vi "laser_constant_current_output_with_DAQ_analog_output.vi"(4 "Exit Refnum":refnum<vi>, 5 "Activate Refnum":refnum<vi>, 7 "VISA resource name":refnum<visa-resource-name>, 8 "error in (no error)":errorcluster, 9 "Current Refnum":refnum<vi>, 10 "Power Refnum":refnum<vi>, 11 "DAQmx Device":tag) -> (0 "error out":errorcluster)   [LabVIEW 2025, in "tSNIP.lvlib"]
uses:
  tSNIP.lvlib
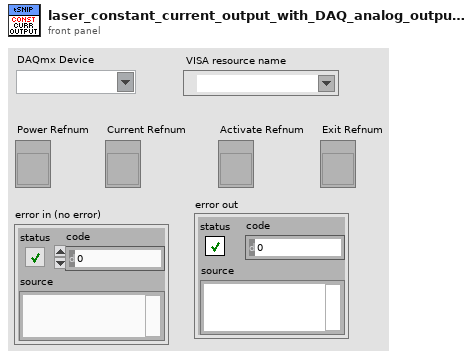
[diagram p1: front panel]
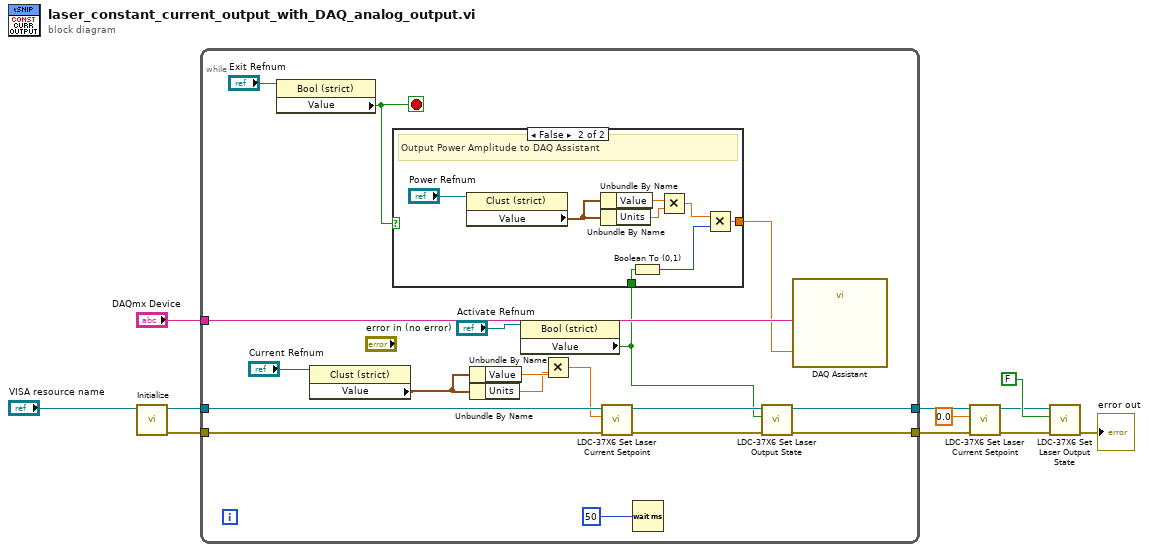
[diagram p0: block diagram]
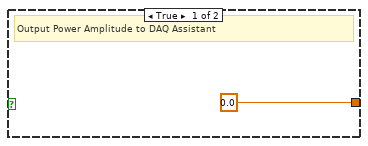
[diagram p2: hidden frame]
diagram:
  n1 = call "Initialize.vi"("VISA resource name"="VISA resource name") -> ("error out"=w9:errorcluster, "VISA resource name out"=w10:refnum<visa-resource-name>)  [unwired: 9 in]
  n2 = while {
    tunnel: w10 -> [w27]
    tunnel: w9 -> [w28]
    tunnel: [w26] -> w8
    tunnel: [w25] -> w7
    tunnel: "DAQmx Device" -> [w22]
    stop <- w12 stop-if-true
    n3 = property class="Bool (strict)"(reference="Exit Refnum") -> ("Value"=w12:bool)  [unwired: 1 in, 2 out]
    n4 = property class="Clust (strict)"(reference="Current Refnum") -> ("Value"=w13:cluster{"Value":dbl, "Units":dbl})  [unwired: 1 in, 2 out]
    n5 = Unbundle By Name(w13) -> ("Value"=w20:dbl)
    n6 = Unbundle By Name(w13) -> ("Units"=w19:dbl)
    n7 = property class="Bool (strict)"(reference="Activate Refnum") -> ("Value"=w16:bool)  [unwired: 1 in, 2 out]
    n8 = case shown="False" w12 {
      tunnel: [0.0 w37] -> w21
      tunnel: w16 -> [_ w33]
      frame True {
        # "Output Power Amplitude to DAQ Assistant"
      }
      frame False {
        # "Output Power Amplitude to DAQ Assistant"
        n9 = property class="Clust (strict)"(reference="Power Refnum") -> ("Value"=w32:cluster{"Value":dbl, "Units":dbl})  [unwired: 1 in, 2 out]
        n10 = Unbundle By Name(w32) -> ("Value"=w36:dbl)
        n11 = Unbundle By Name(w32) -> ("Units"=w35:dbl)
        n12 = Boolean To (0,1)(Boolean=w33) -> (0, 1=w38:i16)
        n13 = Multiply(x=w36, y=w35) -> (x*y=w34:dbl)
        n14 = Multiply(x=w34, y=w38) -> (x*y=w37:dbl)
      }
    }
    n15 = Multiply(x=w20, y=w19) -> (x*y=w18:dbl)
    n16 = call <instrlib>:"LDC-37X6 Set Laser Current Setpoint.vi"("VISA resource name"=w27, "Laser Current Setpoint (A)"=w18, "error in"=w28) -> ("VISA resource name out"=w24:refnum<visa-resource-name>, "error out"=w23:errorcluster)  [unwired: 6 in]
    n17 = Wait (ms)(milliseconds to wait=u32 50) -> ()  [unwired: 1 out]
    n18 = call <instrlib>:"LDC-37X6 Set Laser Output State.vi"("error in"=w23, "Laser Output Enable"=w16, "VISA resource name"=w24) -> ("error out"=w26:errorcluster, "VISA resource name out"=w25:refnum<visa-resource-name>)  [unwired: 7 in]
    n19 = call "DAQ Assistant"("data"=w21, "device name"=w22) -> ()  [unwired: 16 in, 2 out]
  }
  n20 = call <instrlib>:"LDC-37X6 Set Laser Current Setpoint.vi"("VISA resource name"=w7, "Laser Current Setpoint (A)"=0.0, "error in"=w8) -> ("VISA resource name out"=w3:refnum<visa-resource-name>, "error out"=w5:errorcluster)  [unwired: 6 in]
  n21 = call <instrlib>:"LDC-37X6 Set Laser Output State.vi"("error in"=w5, "Laser Output Enable"=FALSE, "VISA resource name"=w3) -> ("error out"=→"error out":errorcluster)  [unwired: 7 in, 1 out]
